vi "Test_API_Write_Raw.vi"() -> ()   [LabVIEW 2021]
uses:
  CANsub_C.lvlib
  api/CANsub_Channel/CANsub_Channel.lvclass
  common/Typedefs/CANsub_connection.ctl
  common/CANsub_Common.lvlib
  common/Typedefs/CANsub_Bit_Rates.ctl
  api/Typedefs/CANsub_Filter.ctl
  api/CANsub_API.lvlib
  api/Typedefs/CANsub_Read_Mode.ctl
  api/Typedefs/CANsub_Ownership.ctl
  api/Typedefs/CANsub_Config.ctl
  api/Typedefs/CANsub_State.ctl
  common/Typedefs/Bit_Timing.ctl
  api/Typedefs/CANsub_Status.ctl
panel:
  out "error out":errorcluster
  out "status tx":T1
  out "ids":u32[](array[numeric]) format="%.0x"
  out "frames received":i32
  in  "rx channel":u8=2
  in  "tx channel":u8=1
  in  "config":T4={"connection"={"host"="192.168.0.49", "channel"=2, "cert path"=path "/home/lvuser/cansub_root_cert.crt"}, "bit rates"={"nominal bit rate"=500000, "nominal sample point"=80.0, "data bit rate"=2000000, "data sample point"=80.0}, "listen only"=FALSE, "filters"=[], "read mode"=enum."Poll", "max bytes per read"=4096, "reader FIFO depth"=0, "reader priority"=0, "ownership"=enum."Direct"} {"filters"."f2" format="%.0x"; "filters"."f1" format="%.0x"}
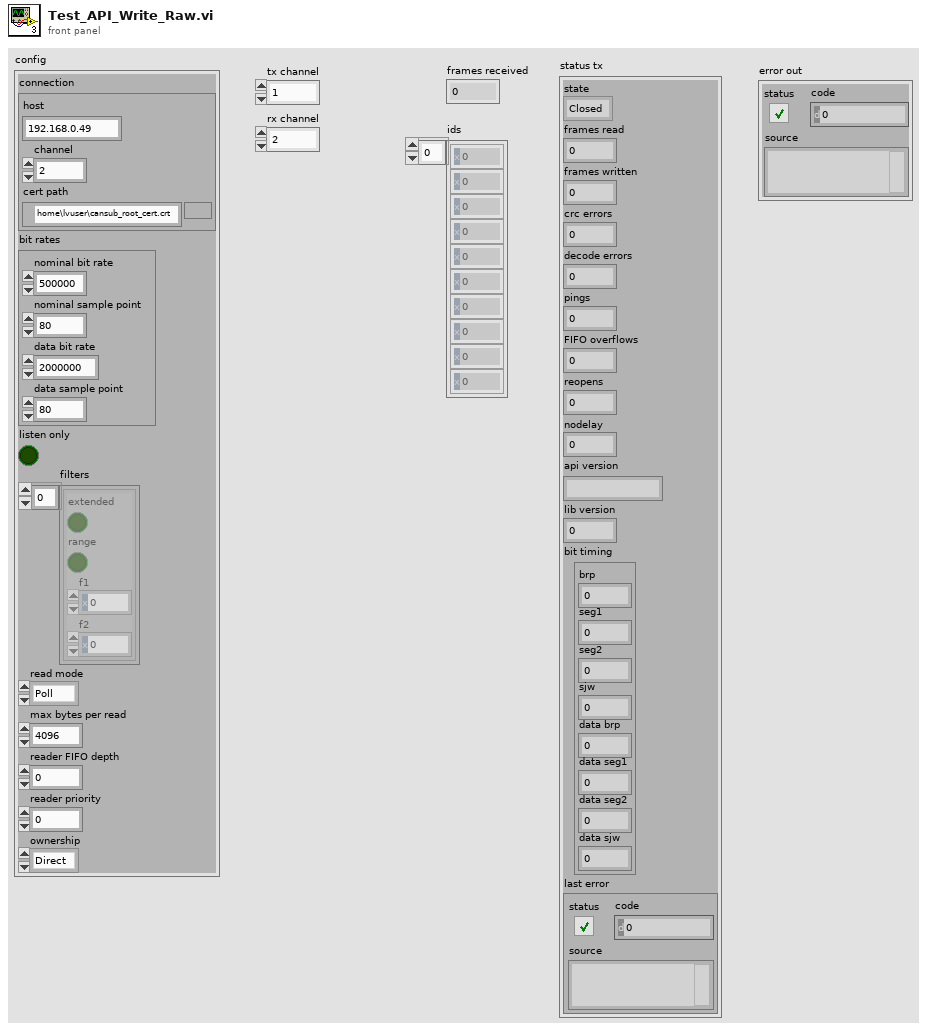
[diagram p1: front panel]
types:
  T1 = typedef "CANsub_API.lvlib/CANsub_Status.ctl" = cluster{"state":T2, "frames read":u32, "frames written":u32, "crc errors":u32, "decode errors":i32, "pings":u32, "FIFO overflows":u32, "reopens":u32, "nodelay":i32, "api version":string, "lib version":u32, "bit timing":T3, "last error":errorcluster}
  T2 = typedef "CANsub_API.lvlib/CANsub_State.ctl" = enum16{"Closed", "Open", "Lost"}
  T3 = typedef "CANsub_Common.lvlib/Bit_Timing.ctl" = cluster{"brp":u16, "seg1":u16, "seg2":u16, "sjw":u16, "data brp":u16, "data seg1":u16, "data seg2":u16, "data sjw":u16}
  T4 = typedef "CANsub_API.lvlib/CANsub_Config.ctl" = cluster{"connection":T5, "bit rates":T6, "listen only":bool, "filters":T7[], "read mode":T8, "max bytes per read":i32, "reader FIFO depth":i32, "reader priority":i32, "ownership":T9}
  T5 = typedef "CANsub_Common.lvlib/CANsub_connection.ctl" = cluster{"host":string, "channel":u8, "cert path":path}
  T6 = typedef "CANsub_Common.lvlib/CANsub_Bit_Rates.ctl" = cluster{"nominal bit rate":u32, "nominal sample point":dbl, "data bit rate":u32, "data sample point":dbl}
  T7 = typedef "CANsub_API.lvlib/CANsub_Filter.ctl" = cluster{"extended":bool, "range":bool, "f1":u32, "f2":u32}
  T8 = typedef "CANsub_API.lvlib/CANsub_Read_Mode.ctl" = enum16{"Poll", "Reader"}
  T9 = typedef "CANsub_API.lvlib/CANsub_Ownership.ctl" = enum16{"Direct", "Shared"}
  T10 = typedef "CANsub_API.lvlib/CANsub_Frames.ctl" = cluster{"count":i32, "t_dev":dbl[], "id":u32[], "flags":u16[], "dlc":u8[], "data len":u8[], "data":u8[]}
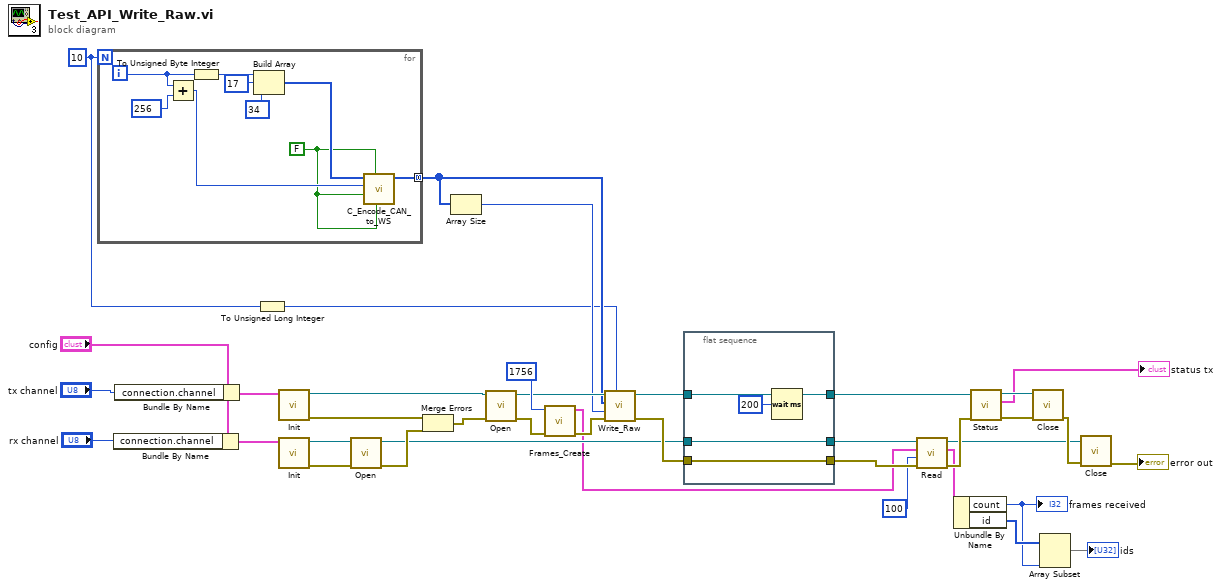
[diagram p0: block diagram]
diagram:
  w10 = 10
  n1 = for {
    N: w10 -> [_]
    tunnel: [w42] -> w11 mode=concatenating
    i -> [w45]
    w39 = FALSE ("ide")
    n2 = Add(x=w45, y=u32 256) -> (x+y=w41:u32)
    n3 = To Unsigned Byte Integer(number=w45) -> (unsigned 8bit integer=w46:u8)
    n4 = Build Array(w46, u8 17 ("element"), u8 34 ("element")) -> (w40:u8[])
    n5 = call "C_Encode_CAN_to_WS.vi"("brs"=w39, "ide"=w39, "fdf"=w39, "id"=w41, "data"=w40) -> ("ws frame"=w42:u8[])  [unwired: 5 in, 1 out]
  }
  n6 = Bundle By Name(cluster="config", "connection.channel"="rx channel") -> (w34:T4)
  n7 = Bundle By Name(cluster="config", "connection.channel"="tx channel") -> (w35:T4)
  n8 = To Unsigned Long Integer(number=w10) -> (unsigned 32bit integer=w9:u32)
  n9 = call "Init.vi"("config"=w35) -> ("error out"=w29:errorcluster, "channel out"=w31:refnum<class "CANsub_Channel.lvclass">)  [unwired: 8 in, 1 out]
  n10 = call "Init.vi"("config"=w34) -> ("error out"=w33:errorcluster, "channel out"=w32:refnum<class "CANsub_Channel.lvclass">)  [unwired: 8 in, 1 out]
  n11 = call-dynamic "Open.vi"("error in (no error)"=w33, "channel in"=w32) -> ("error out"=w30:errorcluster, "channel out"=w15:refnum<class "CANsub_Channel.lvclass">)  [unwired: 8 in]
  n12 = Merge Errors(w29, w30) -> (w28:errorcluster)
  n13 = Array Size(array=w11) -> (size(s)=w12:i32)
  n14 = call-dynamic "Open.vi"("error in (no error)"=w28, "channel in"=w31) -> ("error out"=w27:errorcluster, "channel out"=w19:refnum<class "CANsub_Channel.lvclass">)  [unwired: 8 in]
  n15 = call "Frames_Create.vi"("error in (no error)"=w27, "capacity"=1756) -> ("error out"=w25:errorcluster, "frames"=w8:T10)  [unwired: 8 in]
  n16 = call-dynamic "Write_Raw.vi"("n frames"=w9, "error in (no error)"=w25, "length"=w12, "bytes in"=w11, "channel in"=w19) -> ("error out"=w23:errorcluster, "channel out"=w17:refnum<class "CANsub_Channel.lvclass">)  [unwired: 4 in, 1 out]
  n17 = flat-sequence {
    tunnel: [w50] -> w24
    tunnel: w23 -> [w50]
    tunnel: [w49] -> w18
    tunnel: w17 -> [w49]
    tunnel: [w48] -> w16
    tunnel: w15 -> [w48]
    frame #0 {
      n18 = Wait (ms)(milliseconds to wait=u32 200) -> ()  [unwired: 1 out]
    }
  }
  n19 = call-dynamic "Read.vi"("error in (no error)"=w24, "timeout ms"=100, "frames in"=w8, "channel in"=w16) -> ("error out"=w22:errorcluster, "frames out"=w7:T10, "channel out"=w14:refnum<class "CANsub_Channel.lvclass">)  [unwired: 5 in]
  n20 = Unbundle By Name(w7) -> ("count"=w4:i32, "id"=w5:u32[])
  "frames received" <- w4
  n21 = call-dynamic "Status.vi"("error in (no error)"=w22, "channel in"=w18) -> ("error out"=w21:errorcluster, "status"=→"status tx":T1, "channel out"=w13:refnum<class "CANsub_Channel.lvclass">)  [unwired: 7 in]
  n22 = call-dynamic "Close.vi"("error in (no error)"=w21, "channel in"=w13) -> ("error out"=w20:errorcluster)  [unwired: 8 in, 1 out]
  n23 = Array Subset(array=w5, length=w4) -> (→"ids":u32[])  [unwired: 1 in]
  n24 = call-dynamic "Close.vi"("error in (no error)"=w20, "channel in"=w14) -> ("error out"=→"error out":errorcluster)  [unwired: 8 in, 1 out]
